vi "Lab3_Read_From_File.vi"(8 "error in":errorcluster, 11 "File Path":path) -> (0 "error out":errorcluster, 2 "Array":dbl[](array[numeric]), 3 "Array 2":timestamp[](array[timestamp]))   [LabVIEW 2025]
uses:
  <vilib>/Utility/file.llb/Read Delimited Spreadsheet (string).vi
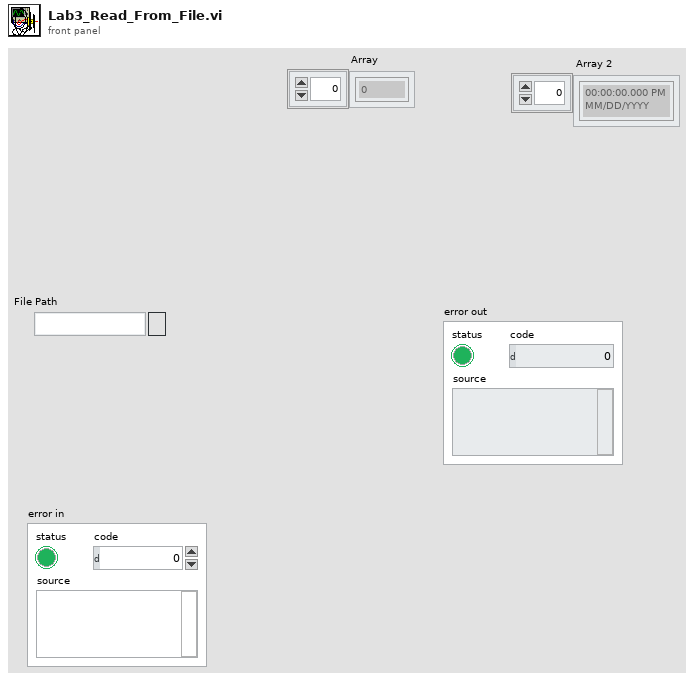
[diagram p1: front panel]
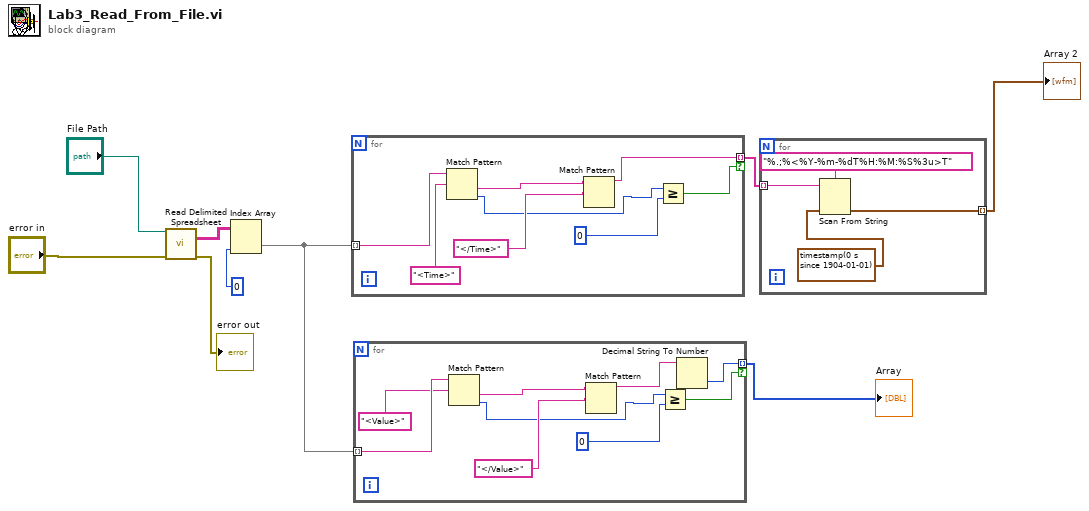
[diagram p0: block diagram]
diagram:
  n1 = call-poly <vilib>:"Read Delimited Spreadsheet.vi"("file path (dialog if empty)"="File Path", "error in (no error)"="error in") -> ("all rows"=w6:string[][], "error out"=→"error out":errorcluster)  [unwired: 8 in, 4 out]
  n2 = Index Array(array=w6, index (col)=0) -> (element=w4:string[])  [unwired: 1 in]
  n3 = for {
    tunnel: w4 -> [w17] mode=indexing
    tunnel: [w10] -> w3 mode=indexing if=w12
    n4 = Match Pattern(string=w17, regular expression="<Time>") -> (after substring=w11:string, offset past match=w14:i32)  [unwired: 1 in, 2 out]
    n5 = Match Pattern(string=w11, regular expression="</Time>") -> (before substring=w10:string)  [unwired: 1 in, 3 out]
    n6 = Greater Or Equal?(x=w14, y=0) -> (x >= y?=w12:bool)
  }
  n7 = for {
    tunnel: w4 -> [w26] mode=indexing
    tunnel: [w18] -> w1 mode=indexing if=w21
    n8 = Match Pattern(string=w26, regular expression="<Value>") -> (after substring=w20:string, offset past match=w23:i32)  [unwired: 1 in, 2 out]
    n9 = Match Pattern(string=w20, regular expression="</Value>") -> (before substring=w19:string)  [unwired: 1 in, 3 out]
    n10 = Greater Or Equal?(x=w23, y=0) -> (x >= y?=w21:bool)
    n11 = Decimal String To Number(string=w19) -> (number=w18:i32)  [unwired: 2 in, 1 out]
  }
  "Array" <- w1
  n12 = for {
    tunnel: w3 -> [w30] mode=indexing
    tunnel: [w27] -> w2 mode=indexing
    n13 = Scan From String(format string="%.;%<%Y-%m-%dT%H:%M:%S%3u>T", input string=w30, default 1=timestamp(0 s since 1904-01-01)) -> (output 1=w27:timestamp)  [unwired: 2 in, 3 out]
  }
  "Array 2" <- w2
